vi "Read U8 External Payload.vi"(8 "error in (no error)":errorcluster, 9 "Timeout (ms)":i32=100, 10 "Data in":u8[](array[numeric]), 11 "CIF_Iceoryx_PCAP_Universal in":refnum<class "CIF_Iceoryx_PCAP_Universal.lvclass">) -> (0 "error out":errorcluster, 1 "timed out?":bool, 2 "Data out":u8[](array[numeric]), 3 "CIF_Iceoryx_PCAP_Universal out":refnum<class "CIF_Iceoryx_PCAP_Universal.lvclass">, 4 "Header":T1)   [LabVIEW 2021, in "CIF_Iceoryx_PCAP_Universal.lvclass"]
doc: "Read the full payload bytes, including the encoded header. This is intended for advanced applications where the full buffer will be sent externally. The Data in size must match the size of the full payload capacity."
uses:
  CIF_Iceoryx_PCAP_Universal.lvclass
  D:/dev/Packages/CIF_Channels_Core/src/CIFChannels/CIFChannels.lvclass
  ChannelCommon/typedef/FIFO Header.ctl
  CIFChannels/CIFChannels.lvclass/CIFChannels.ctl
  CIF_Iceoryx_PCAP_Universal.lvclass/CIF_Iceoryx_PCAP_Universal.ctl
  <vilib>/CIF Foundation/CIF Utilities/Statistics/I64/Stats_I64_CIF_U.lvclass/Stats_I64_CIF_U.ctl
  CIFChannels/Accessors/Read Channel State.vi
  CIFChannels/Accessors/Read Direction.vi
  <vilib>/CIF Foundation/CIF Iceoryx/SubVIs/Get Path.vi
  <vilib>/CIF Foundation/CIF Iceoryx/SubVIs/Convert Error.vi
  <vilib>/CIF Foundation/CIF Iceoryx/Refnum/CIF Subscriber from Refnum.vi
  <vilib>/CIF Foundation/CIF Utilities/DataTypes/Flatten Unflatten/Unflatten U64.vi
  <vilib>/CIF Foundation/CIF Utilities/DataTypes/Flatten Unflatten/Unflatten I64.vi
  ChannelCommon/Utilities/Add Error.vi
  <vilib>/CIF Foundation/CIF Utilities/Statistics/I64/X1 minus X0.vi
  <vilib>/CIF Foundation/CIF Utilities/Time/System Time/Get System Time.vi
  <vilib>/CIF Foundation/CIF Utilities/Statistics/I64/X1 minus X0.vi/dfabcf33-0dbc-4041-80a5-3dc0c86d2989.vi
  <vilib>/CIF Foundation/CIF Utilities/Statistics/I64/X1 minus X0.vi/dfabcf33-0dbc-4041-80a5-3dc0c86d2989.vi/9eb60a9a-770f-4d2d-8b3f-8465c267ecc9.vi
  <vilib>/CIF Foundation/CIF Iceoryx/SubVIs/Convert Error Core.vi
  ChannelCommon/Utilities/Add Error Core.vi
  ChannelCommon/ChannelCommon.lvlib
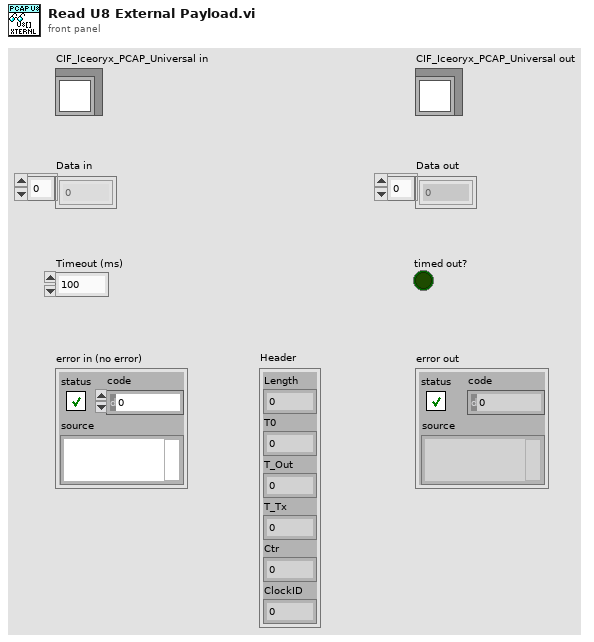
[diagram p1: front panel]
types:
  T1 = typedef "ChannelCommon.lvlib/FIFO Header.ctl" = cluster{"Length":u64, "T0":i64, "T_Out":i64, "T_Tx":i64, "Ctr":u64, "ClockID":u8}
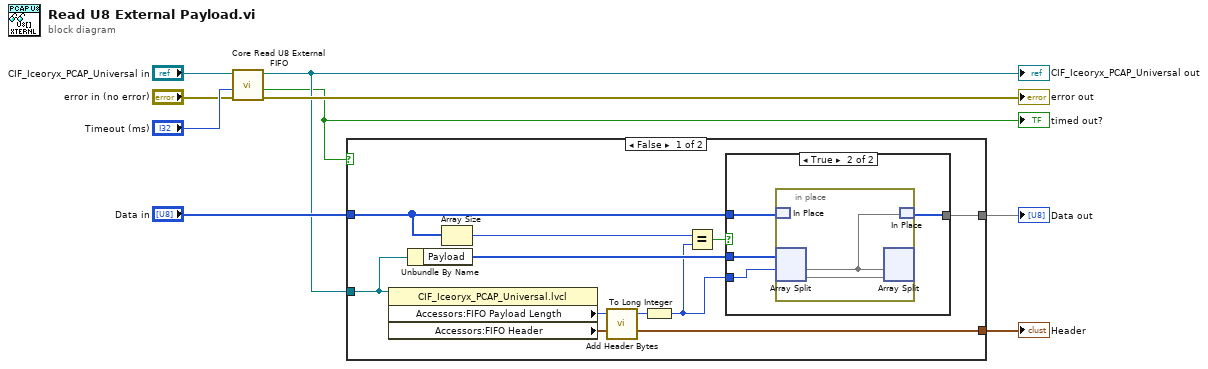
[diagram p0: block diagram]
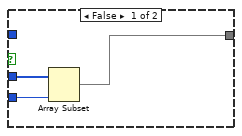
[diagram p2: hidden frame]
diagram:
  n1 = call "Core Read U8 External FIFO.vi"("error in (no error)"="error in (no error)", "Timeout (ms)"="Timeout (ms)", "CIFFIFO in"="CIF_Iceoryx_PCAP_Universal in") -> ("error out"=→"error out":errorcluster, "timed out?"=w1:bool, "CIFFIFO out"=w2:refnum<class "CIF_Iceoryx_PCAP_Universal.lvclass">)  [unwired: 6 in]
  "CIF_Iceoryx_PCAP_Universal out" <- w2
  "timed out?" <- w1
  n2 = case shown="False" w1 {
    tunnel: w2 -> [w19 _]
    tunnel: [w17 w29] -> w7
    tunnel: [w16 _] -> w8
    tunnel: "Data in" -> [w13 w29]
    frame False {
      n3 = property class="CIF_Iceoryx_PCAP_Universal.lvcl"(reference=w19) -> ("Accessors:FIFO Payload Length"=w11:u64, "Accessors:FIFO Header"=w16:T1)  [unwired: 1 in, 2 out]
      n4 = Unbundle By Name(w19) -> ("Payload"=w18:u8[])
      n5 = Array Size(array=w13) -> (size(s)=w15:i32)
      n6 = call "Add Header Bytes.vi"("Bytes/Msg"=w11) -> ("Bytes/Msg with header"=w10:u64)  [unwired: 3 in]
      n7 = To Long Integer(number=w10) -> (32bit integer=w14:i32)
      n8 = Equal?(x=w15, y=w14) -> (x = y?=w12:bool)
      n9 = case shown="True" w12 {
        tunnel: w18 -> [w22 w25]
        tunnel: [w20 w23] -> w17
        tunnel: w14 -> [w21 w24]
        tunnel: w13 -> [_ w26]
        frame False {
          n10 = Array Subset(array=w22, length=w21) -> (w20:u8[])  [unwired: 1 in]
        }
        frame True {
          n11 = in-place {
            n12 = in-place-match #1(w26) -> ()  [unwired: 1 out]
            n13 = in-place-split #2(w25, w24) -> (w27:u8[], w28:u8[])
            n14 = in-place-split #2(w27, w28) -> ()  [unwired: 2 out]
            n15 = in-place-match #1(w27) -> (w23:u8[])
          }
        }
      }
    }
    frame True {
    }
  }
  "Header" <- w8
  "Data out" <- w7
